vi "raspberry_pi_control_panel.vi"() -> ()   [LabVIEW 2026]
uses:
  <userlib>/_OpenG.lib/lvdata/lvdata.llb/openg_variant.lvlib
panel:
  in  "Kill on Stop":bool
  in  "Action":T1(ring)
  in  "Run":bool
  out "Output":string
  out "Command Preview":string
  in  "Wait for Convergence":bool
  in  "Auto Plot":bool
  in  "Auto Logs":bool
  in  "Monitor Seconds":dbl
  in  "Iterations":dbl
  in  "Nodes":string
  in  "Scenario":string
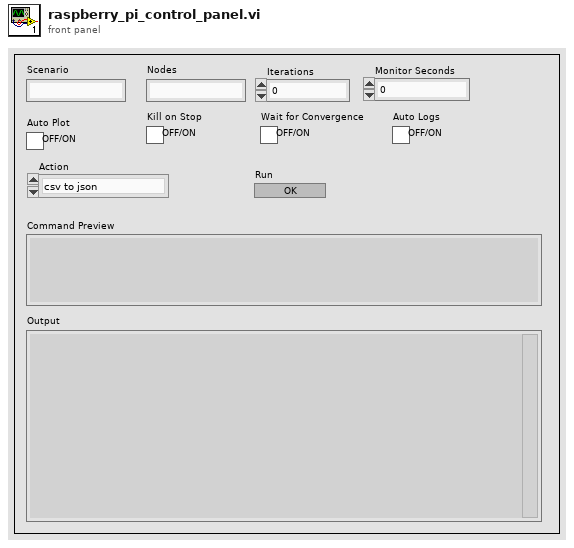
[diagram p1: front panel]
types:
  T1 = enum16{"csv to json", "ping", "deploy", "start", "stop", "monitor", "logs", "centralized-baseline"}
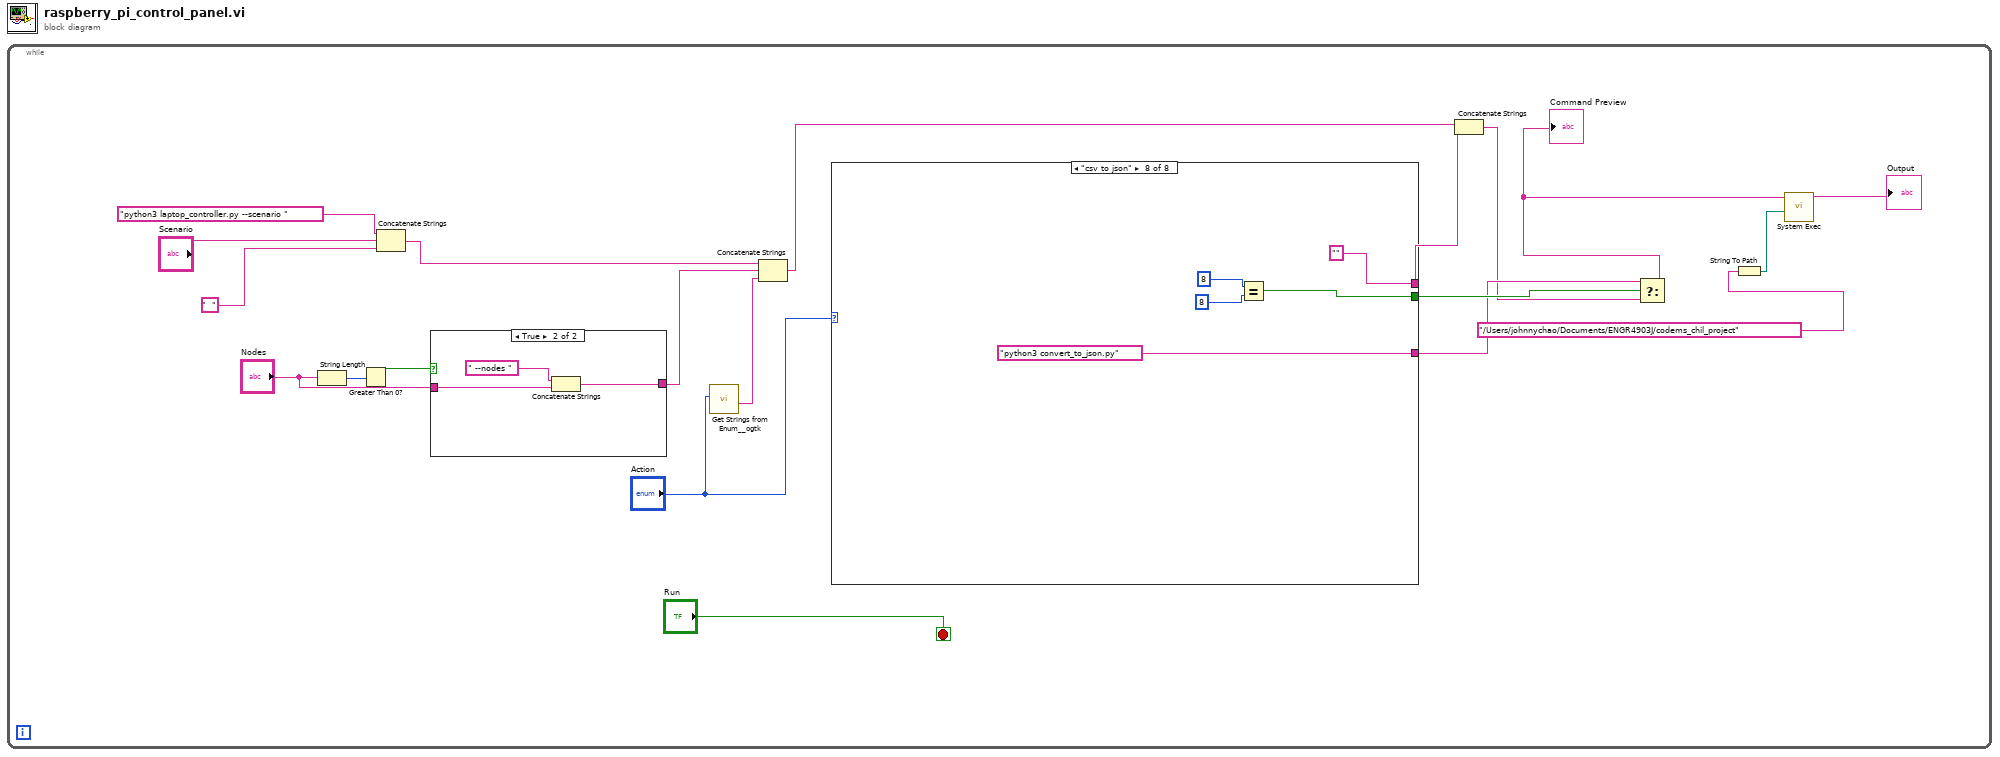
[diagram p0: block diagram]
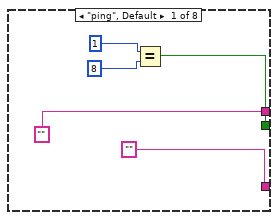
[diagram p2: hidden frame]
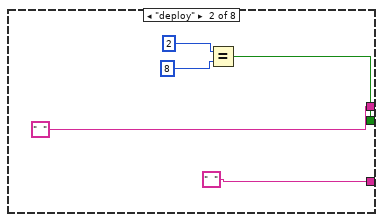
[diagram p3: hidden frame]
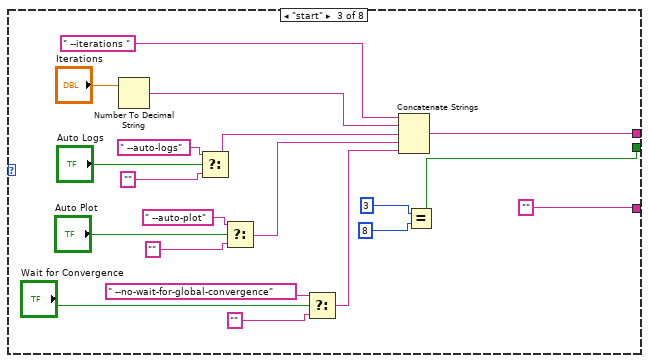
[diagram p4: hidden frame]
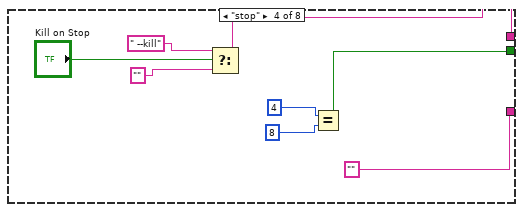
[diagram p5: hidden frame]
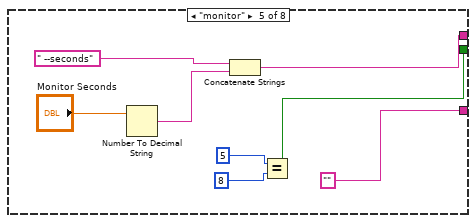
[diagram p6: hidden frame]
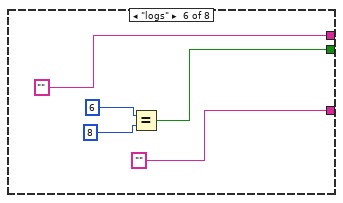
[diagram p7: hidden frame]
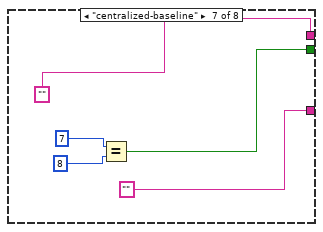
[diagram p8: hidden frame]
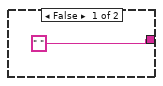
[diagram p9: hidden frame]
diagram:
  n1 = while {
    stop <- "Run" stop-if-true
    n2 = String Length(string="Nodes") -> (length=w16:i32)
    n3 = Greater Than 0?(x=w16) -> (x > 0?=w15:bool)
    n4 = Concatenate Strings("python3 laptop_controller.py --scenario ", "Scenario", "  ") -> (w14:string)
    n5 = case shown="True" w15 {
      tunnel: [" " w84] -> w12
      tunnel: "Nodes" -> [_ w83]
      frame False {
      }
      frame True {
        n6 = Concatenate Strings(" --nodes ", w83) -> (w84:string)
      }
    }
    n7 = call <userlib>:"Get Strings from Enum__ogtk.vi"("Enum"="Action") -> ("String Value"=w5:string)  [unwired: 7 in, 3 out]
    n8 = Concatenate Strings(w14, w12, w5) -> (w9:string)
    n9 = case shown="\"csv to json\"" "Action" {
      tunnel: ["" "  " w35 w55 w63 "" "" ""] -> w10
      tunnel: [w22 w27 w32 w51 w60 w68 w73 w79] -> w4
      tunnel: ["" "  " "" "" "" "" "" "python3 convert_to_json.py"] -> w3
      frame "ping", Default {
        n10 = Equal?(x=1, y=8) -> (x = y?=w22:bool)
      }
      frame "deploy" {
        n11 = Equal?(x=2, y=8) -> (x = y?=w27:bool)
      }
      frame "start" {
        n12 = Number To Decimal String(number="Iterations") -> (decimal integer string=w39:string)  [unwired: 1 in]
        n13 = Select(t=" --auto-logs", s="Auto Logs", f="") -> (s? t:f=w38:string)
        n14 = Select(t=" --auto-plot", s="Auto Plot", f="") -> (s? t:f=w37:string)
        n15 = Select(t=" --no-wait-for-global-convergence", s="Wait for Convergence", f="") -> (s? t:f=w36:string)
        n16 = Concatenate Strings(" --iterations ", w39, w38, w37, w36) -> (w35:string)
        n17 = Equal?(x=3, y=8) -> (x = y?=w32:bool)
      }
      frame "stop" {
        n18 = Select(t=" --kill", s="Kill on Stop", f="") -> (s? t:f=w55:string)
        n19 = Equal?(x=4, y=8) -> (x = y?=w51:bool)
      }
      frame "monitor" {
        n20 = Number To Decimal String(number="Monitor Seconds") -> (decimal integer string=w64:string)  [unwired: 1 in]
        n21 = Concatenate Strings(" --seconds", w64) -> (w63:string)
        n22 = Equal?(x=5, y=8) -> (x = y?=w60:bool)
      }
      frame "logs" {
        n23 = Equal?(x=6, y=8) -> (x = y?=w68:bool)
      }
      frame "centralized-baseline" {
        n24 = Equal?(x=7, y=8) -> (x = y?=w73:bool)
      }
      frame "csv to json" {
        n25 = Equal?(x=8, y=8) -> (x = y?=w79:bool)
      }
    }
    n26 = Concatenate Strings(w9, w10) -> (w2:string)
    n27 = Select(t=w3, s=w4, f=w2) -> (s? t:f=w1:string)
    "Command Preview" <- w1
    n28 = String To Path(string="/Users/johnnychao/Documents/ENGR4903J/codems_chil_project") -> (path=w7:path)
    n29 = call <vilib>:"System Exec.vi"("working directory"=w7, "command line"=w1) -> ("standard output"=→"Output":string)  [unwired: 6 in, 3 out]
  }
